vi "Initialize LUT.vi"(11 "Run ID":string="run-1791786455269") -> (3 "User Events Metadata":T1[](array[typedef]))   [LabVIEW 2026, in "dependencies.lvlib"]
uses:
  dependencies.lvlib
  KeyboardAndMouseDataAcquisition.ctl
  KeyType.ctl
  99a060bb-7a0f-4e6a-9d2d-08bfaee5256b.vi
  <vilib>/JDP Science/JSONtext/JSON text to Variant.vi
  <vilib>/JDP Science/JSONtext/LVClass Serializer/JSONtext LVClass Serializer.lvclass
panel:
  out "Numeric":i32
  out "error out":errorcluster
  out "appended path":path
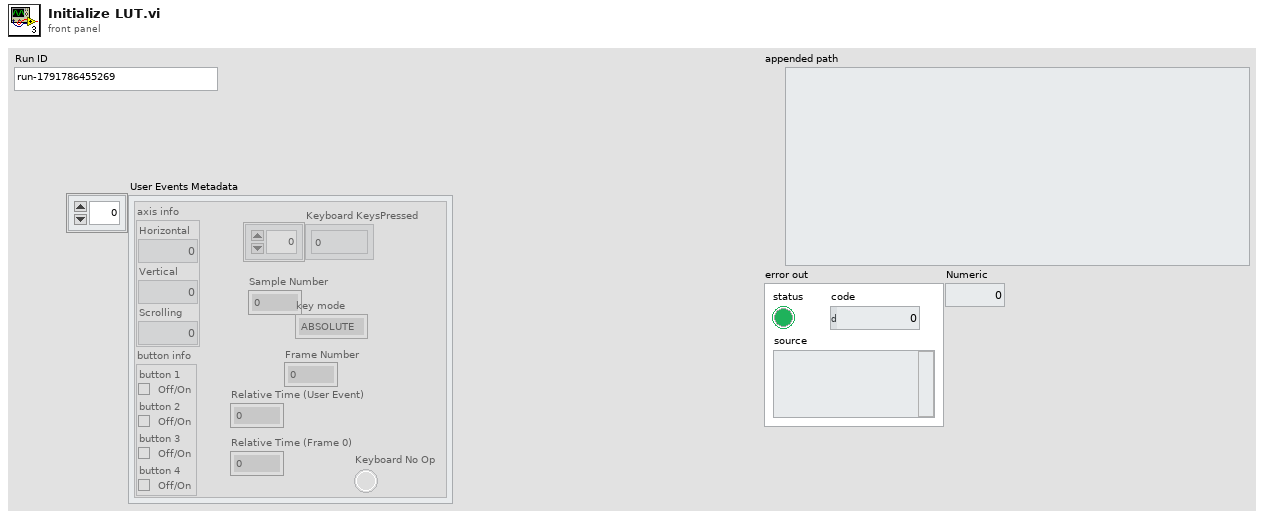
[diagram p1: front panel]
types:
  T1 = typedef "dependencies.lvlib/KeyboardAndMouseDataAcquisition.ctl" = cluster{"axis info":cluster{"Horizontal":i32, "Vertical":i32, "Scrolling":i32}, "button info":cluster{"button 1":bool, "button 2":bool, "button 3":bool, "button 4":bool}, "Relative Time (User Event)":dbl, "Sample Number":u32, "Relative Time (Frame 0)":dbl, "key mode":enum16{"RELATIVE", "ABSOLUTE"}, "Frame Number":u32, "Keyboard KeysPressed":T2[], "Keyboard No Op":bool}
  T2 = typedef "dependencies.lvlib/KeyType.ctl" = enum16{"0", "1", "2", "3", "4", "5", "6", "7", "8", "9", "A", "B", "C", "D", "E", "F", "G", "H", "I", "J", "K", "L", "M", "N", "O", "P", "Q", "R", "S", "T", "U", "V", "W", "X", "Y", "Z", "F1", "F2", "F3", "F4", "F5", "F6", "F7", "F8", "F9", "F10", "F11", "F12", "F13", "F14", "F15", "ADD", "BACK", "BACKSLASH", "CAPITAL", "COMMA", "DECIMAL", "DELETE", "DIVIDE", "DOWN", "END", "EQUALS", "ESCAPE", "GRAVE (`)", "HOME", "INSERT", "LBRACKET", "LCONTROL", "LEFT", "L ALT", "LSHIFT", "LWIN", "MINUS", "MULTIPLY", "NEXT", "NUMLOCK", "NUMPAD_0", "NUMPAD_1", "NUMPAD_2", "NUMPAD_3", "NUMPAD_4", "NUMPAD_5", "NUMPAD_6", "NUMPAD_7", "NUMPAD_8", "NUMPAD_9", "PAUSE", "PERIOD", "PRIOR (PG UP)", "RBRACKET", "RCONTROL", "RETURN", "RIGHT", "R ALT", "RSHIFT", "RWIN", "SCROLL", "SEMICOLON", "SLASH", "SPACE", "SUBTRACT", "TAB", "UP", "ENTER (num pad)", "' (quote)"}
  T3 = enum16{"0", "1", "2", "3", "4", "5", "6", "7", "8", "9", "A", "B", "C", "D", "E", "F", "G", "H", "I", "J", "K", "L", "M", "N", "O", "P", "Q", "R", "S", "T", "U", "V", "W", "X", "Y", "Z", "F1", "F2", "F3", "F4", "F5", "F6", "F7", "F8", "F9", "F10", "F11", "F12", "F13", "F14", "F15", "ADD", "BACK", "BACKSLASH", "CAPITAL", "COMMA", "DECIMAL", "DELETE", "DIVIDE", "DOWN", "END", "EQUALS", "ESCAPE", "GRAVE (`)", "HOME", "INSERT", "LBRACKET", "LCONTROL", "LEFT", "L ALT", "LSHIFT", "LWIN", "MINUS", "MULTIPLY", "NEXT", "NUMLOCK", "NUMPAD_0", "NUMPAD_1", "NUMPAD_2", "NUMPAD_3", "NUMPAD_4", "NUMPAD_5", "NUMPAD_6", "NUMPAD_7", "NUMPAD_8", "NUMPAD_9", "PAUSE", "PERIOD", "PRIOR (PG UP)", "RBRACKET", "RCONTROL", "RETURN", "RIGHT", "R ALT", "RSHIFT", "RWIN", "SCROLL", "SEMICOLON", "SLASH", "SPACE", "SUBTRACT", "TAB", "UP", "ENTER (num pad)", "' (quote)"}[]
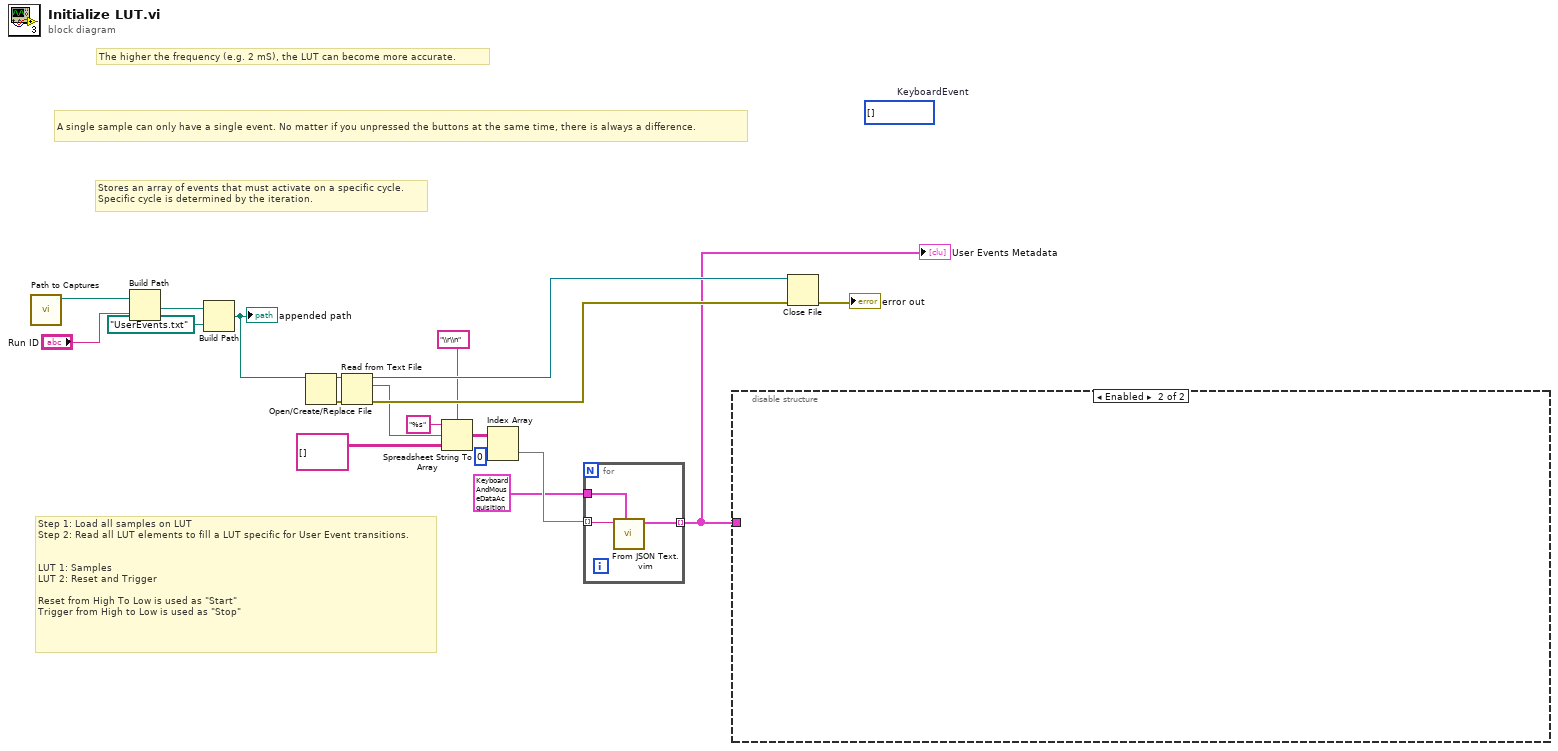
[diagram p0: block diagram]
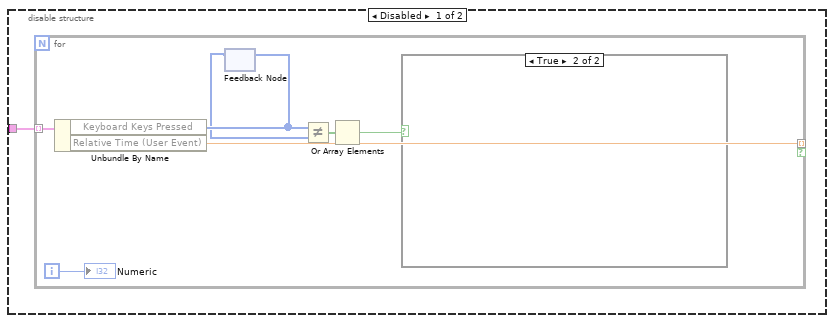
[diagram p2: hidden frame]
diagram:
  (unwired) T2[] [] items=["0", "1", "2", "3", "4", "5", "6", "7", "8", "9", "A", "B", "C", "D", "E", "F", "G", "H", "I", "J", "K", "L", "M", "N", "O", "P", "Q", "R", "S", "T", "U", "V", "W", "X", "Y", "Z", "F1", "F2", "F3", "F4", "F5", "F6", "F7", "F8", "F9", "F10", "F11", "F12", "F13", "F14", "F15", "ADD", "BACK", "BACKSLASH", "CAPITAL", "COMMA", "DECIMAL", "DELETE", "DIVIDE", "DOWN", "END", "EQUALS", "ESCAPE", "GRAVE (`)", "HOME", "INSERT", "LBRACKET", "LCONTROL", "LEFT", "L ALT", "LSHIFT", "LWIN", "MINUS", "MULTIPLY", "NEXT", "NUMLOCK", "NUMPAD_0", "NUMPAD_1", "NUMPAD_2", "NUMPAD_3", "NUMPAD_4", "NUMPAD_5", "NUMPAD_6", "NUMPAD_7", "NUMPAD_8", "NUMPAD_9", "PAUSE", "PERIOD", "PRIOR (PG UP)", "RBRACKET", "RCONTROL", "RETURN", "RIGHT", "R ALT", "RSHIFT", "RWIN", "SCROLL", "SEMICOLON", "SLASH", "SPACE", "SUBTRACT", "TAB", "UP", "ENTER (num pad)", "' (quote)"]  # KeyboardEvent
  # "Step 1: Load all samples on LUT\nStep 2: Read all LUT elements to fill a LUT specific for User Event transitions.\n\n\nLUT 1: Samples\nLUT 2: Reset and Trigger\n\nReset from High To Low is used as \"Start\"\nTrigger from High to Low is used as \"Stop\""
  # "The higher the frequency (e.g. 2 mS), the LUT can become more accurate."
  # "Stores an array of events that must activate on a specific cycle.\nSpecific cycle is determined by the iteration."
  # "A single sample can only have a single event. No matter if you unpressed the buttons at the same time, there is always a difference."
  n1 = call "Path to Captures.vi"() -> ("Captures"=w19:path)  [unwired: 11 in]
  n2 = Build Path(base path=w19, name or relative path="Run ID") -> (appended path=w17:path)
  n3 = Build Path(base path=w17, name or relative path=path "UserEvents.txt") -> (appended path=w2:path)
  "appended path" <- w2
  n4 = Open/Create/Replace File(file path (use dialog)=w2) -> (refnum out=w13:refnum<file>, error out=w15:errorcluster)  [unwired: 5 in, 1 out]
  n5 = Read from Text File(file (use dialog)=w13, error in=w15) -> (refnum out=w12:refnum<file>, text=w9:string, error out=w14:errorcluster)  [unwired: 2 in, 1 out]
  n6 = Spreadsheet String To Array(delimiter (Tab)="\\r\\n", format string="%s", spreadsheet string=w9, array type (2D Dbl)=string[][] [] ("text")) -> (array=w6:string[][])
  n7 = Index Array(array=w6, index (col)=0 ("disabled index (col)")) -> (element=w4:string[])  [unwired: 1 in]
  n8 = for {
    tunnel: w4 -> [w22] mode=indexing
    tunnel: [w21] -> w1 mode=indexing
    tunnel: T1 {"axis info"={"Horizontal"=0, "Vertical"=0, "Scrolling"=0}, "button info"={"button 1"=FALSE, "button 2"=FALSE, "button 3"=FALSE, "button 4"=FALSE}, "Relative Time (User Event)"=0.0, "Sample Number"=0, "Relative Time (Frame 0)"=0.0, "key mode"=enum."ABSOLUTE", "Frame Number"=0, "Keyboard KeysPressed"=[], "Keyboard No Op"=FALSE} ("KeyboardAndMouseData") -> [w20]
    n9 = call "From JSON Text.vim"("Data Type and Default Value"=w20, "JSON"=w22) -> ("Data out"=w21:T1)  [unwired: 8 in, 1 out]
  }
  "User Events Metadata" <- w1
  n10 = disable-structure shown="Enabled" {
    disable-tunnel: w1 -> [w23 _]
    frame Disabled {
      n11 = for {
        tunnel: w23 -> [w30] mode=indexing
        tunnel: [w26] -> _ mode=indexing if=_
        i -> [w25]
        n12 = Unbundle By Name(w30) -> ("Keyboard Keys Pressed"=w29:T3, "Relative Time (User Event)"=w26:dbl)
        n13 = feedback-in #1(w29) -> ()
        n14 = feedback #1() -> (w28:T3)  [unwired: 1 in]
        n15 = Not Equal?(x=w29, y=w28) -> (x != y?=w27:bool[])
        n16 = Or Array Elements(Boolean array=w27) -> (logical OR=w24:bool)
        n17 = case shown="True" w24 {
          frame False {
          }
          frame True {
          }
        }
        "Numeric" <- w25
      }
    }
    frame Enabled {
    }
  }
  n18 = Close File(refnum=w12, error in=w14) -> (error out=→"error out":errorcluster)  [unwired: 1 out]
